vi "List ARNs Recursive.vi"(8 "error in (no error)":errorcluster, 10 "NextToken":string, 11 "ARN in":refnum<class "ARN.lvclass">) -> (0 "error out":errorcluster, 3 "ARNs out":refnum<class "ARN.lvclass">[](array[class]))   [LabVIEW 2015, in "NI_AWS_Core.lvlib" / "ARN.lvclass"]
uses:
  ARN.lvclass
  HTTP Request/HTTP Request.lvclass
  HTTP Request/Name Value Pair.ctl
  HTTP Request/Request Options.ctl
  XML Parsing/NI_XML Parsing.lvlib
  HTTP Request/URL formatting.ctl
  HTTP Request/Region handling.ctl
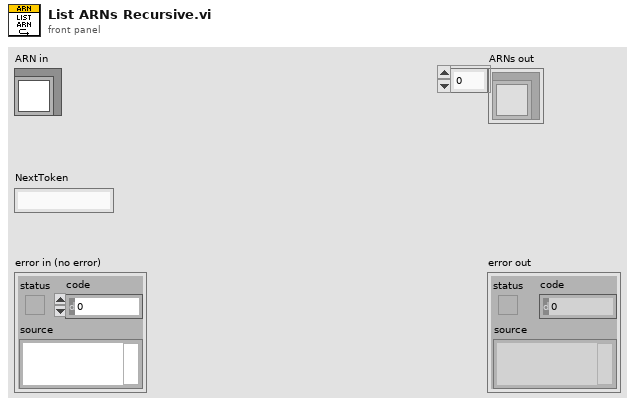
[diagram p1: front panel]
types:
  T1 = typedef "NI_AWS_Core.lvlib/HTTP Request.lvclass/Name Value Pair.ctl" = cluster{"name":string, "value":string}
  T2 = typedef "NI_AWS_Core.lvlib/HTTP Request.lvclass/Request Options.ctl" = cluster{"request headers":T1[], "request parameters":T1[], "request body":string, "region handling":T3, "URL formatting":T4}
  T3 = typedef "NI_AWS_Core.lvlib/HTTP Request.lvclass/Region handling.ctl" = enum16{"use region everywhere", "use region (authentication only)", "use region (URL only)", "ignore region everwhere"}
  T4 = typedef "NI_AWS_Core.lvlib/HTTP Request.lvclass/URL formatting.ctl" = enum16{"region-", "region."}
  T5 = typedef "NI_AWS_Core.lvlib/HTTP Request.lvclass/Response.ctl" = cluster{"Headers":string, "Body":string}
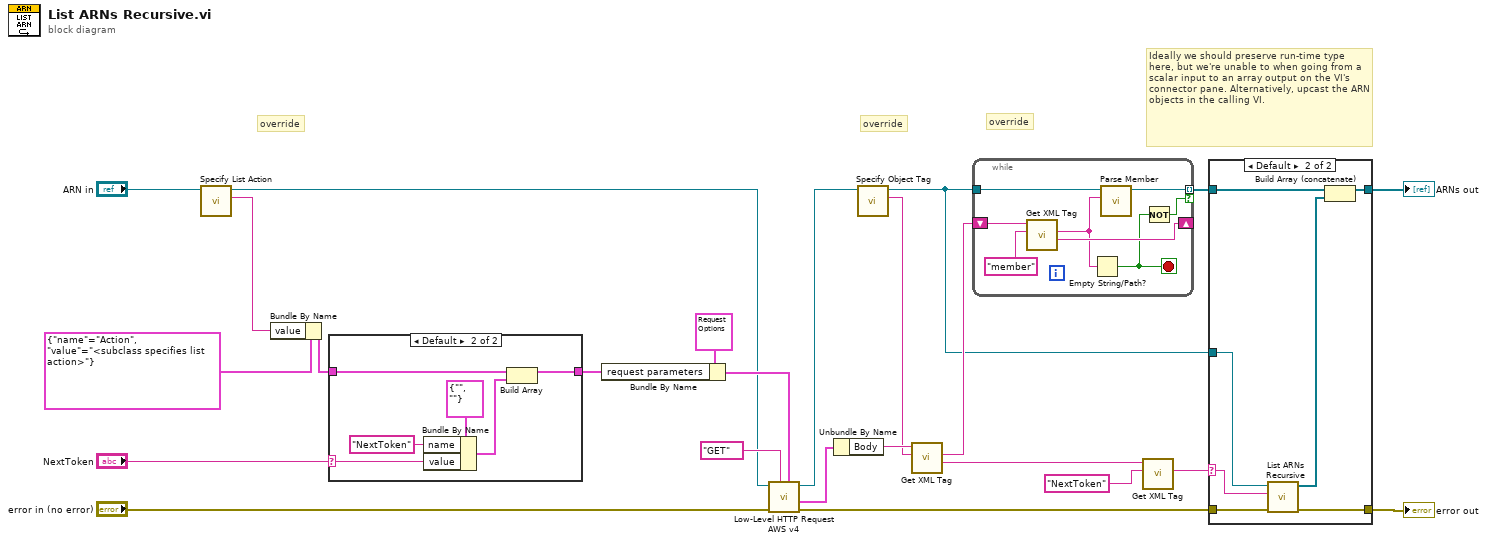
[diagram p0: block diagram]
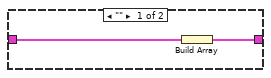
[diagram p3: hidden frame]
diagram:
  # "override"
  # "Ideally we should preserve run-time type here, but we're unable to when going from a scalar input to an array output on the VI's connector pane. Alternatively, upcast the ARN objects in the calling VI."
  # "override"
  # "override"
  n1 = call-dynamic "Specify List Action.vi"("ARN in"="ARN in") -> ("List Action"=w9:string, "ARN out"=w2:refnum<class "ARN.lvclass">)  [unwired: 9 in]
  n2 = Bundle By Name(cluster=T1 {"name"="Action", "value"="<subclass specifies list action>"} ("Cluster"), "value"=w9) -> (w10:T1)
  n3 = case shown="Default" "NextToken" {
    selector: "NextToken" -> [_ w27]
    tunnel: w10 -> [w26 w32]
    tunnel: [w25 w28] -> w20
    frame "" {
      n4 = Build Array(w26) -> (w25:T1[])
    }
    frame Default {
      n5 = Bundle By Name(cluster=T1 {"name"="", "value"=""} ("element"), "name"="NextToken", "value"=w27) -> (w29:T1)
      n6 = Build Array(w32, w29) -> (w28:T1[])
    }
  }
  n7 = Bundle By Name(cluster=T2 {"request headers"=[], "request parameters"=[{"name"="Action", "value"="ListQueues"}], "request body"="", "region handling"=enum."use region everywhere", "URL formatting"=enum."region."} ("Request Options"), "request parameters"=w20) -> (w7:T2)
  n8 = call "Low-Level HTTP Request AWS v4.vi"("Request Options"=w7, "HTTP-Verb"="GET", "error in (no error)"="error in (no error)", "AWS Core in"=w2) -> ("error out"=w19:errorcluster, "Response"=w5:T5, "AWS Core out"=w1:refnum<class "ARN.lvclass">)  [unwired: 4 in, 1 out]
  n9 = Unbundle By Name(w5) -> ("Body"=w14:string)
  n10 = call-dynamic "Specify Object Tag.vi"("ARN in"=w1) -> ("Object tag"=w8:string, "ARN out"=w3:refnum<class "ARN.lvclass">)  [unwired: 9 in]
  n11 = call "Get XML Tag.vi"("Tag name"=w8, "XML String in"=w14) -> ("Remaining string"=w13:string, "Tag value"=w15:string)  [unwired: 5 in, 3 out]
  n12 = while {
    shift-right: [w39] -> _
    shift-left: w15 -> [w40]
    tunnel: w3 -> [w35]
    tunnel: [w34] -> w12 mode=indexing if=w36
    stop <- w37 stop-if-true
    n13 = call "Get XML Tag.vi"("Tag name"="member", "XML String in"=w40) -> ("Remaining string"=w39:string, "Tag value"=w33:string)  [unwired: 5 in, 3 out]
    n14 = Empty String/Path?(string/path=w33) -> (empty?=w37:bool)
    n15 = call-dynamic "Parse Member.vi"("member"=w33, "ARN in"=w35) -> ("ARN out"=w34:refnum<class "ARN.lvclass">)  [unwired: 8 in, 1 out]
    n16 = Not(x=w37) -> (.not. x?=w36:bool)
  }
  n17 = call "Get XML Tag.vi"("Tag name"="NextToken", "XML String in"=w13) -> ("Tag value"=w17:string)  [unwired: 5 in, 4 out]
  n18 = case shown="Default" w17 {
    selector: w17 -> [_ w44]
    tunnel: w19 -> [w42 w49]
    tunnel: [w42 w48] -> w18
    tunnel: w12 -> [w41 w47]
    tunnel: [w41 w45] -> w16
    tunnel: w3 -> [_ w43]
    frame "" {
    }
    frame Default {
      n19 = call "List ARNs Recursive.vi"("error in (no error)"=w49, "NextToken"=w44, "ARN in"=w43) -> ("error out"=w48:errorcluster, "ARNs out"=w46:refnum<class "ARN.lvclass">[])  [unwired: 7 in]
      n20 = Build Array (concatenate)(w47, w46) -> (w45:refnum<class "ARN.lvclass">[])
    }
  }
  "error out" <- w18
  "ARNs out" <- w16
